vi "update event timing.vi"(4 "update duration":bool, 6 "Duration (s)":dbl, 8 "Start Time":timestamp format="%<%x %.3X>T", 9 "set start to now":bool, 10 "update start":bool, 11 "event":refnum<class "event.lvclass">) -> (0 "error out":errorcluster, 3 "updated event":refnum<class "event.lvclass">)   [LabVIEW 2020, in "nominal core steps.lvlib"]
doc: "Change the start time and duration of the event. Use flags to indicate which actions to take."
uses:
  nominal core steps.lvlib
  <vilib>/Nominal/Nominal IO Client/lv_src/event/event.lvclass
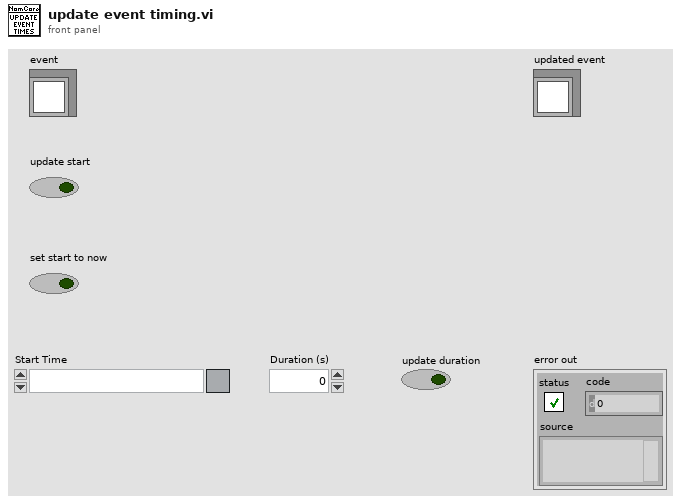
[diagram p1: front panel]
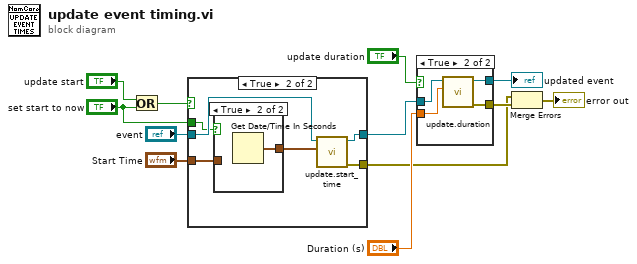
[diagram p0: block diagram]
diagram:
  n1 = Or(x="update start", y="set start to now") -> (x .or. y?=w2:bool)
  n2 = case shown="True" w2 {
    tunnel: [w13 w19] -> w6
    tunnel: [_ w18] -> w7
    tunnel: "event" -> [w13 w17]
    tunnel: "Start Time" -> [_ w14]
    tunnel: "set start to now" -> [_ w16]
    frame False {
    }
    frame True {
      n3 = case shown="True" w16 {
        tunnel: [w20 w21] -> w15
        tunnel: w14 -> [w20 _]
        frame False {
        }
        frame True {
          n4 = Get Date/Time In Seconds() -> (seconds since 1Jan1904=w21:timestamp)
        }
      }
      n5 = call <vilib>:"update.start_time.vi"("Start Time (empty: now)"=w15, "event in"=w17) -> ("error out"=w18:errorcluster, "event out"=w19:refnum<class "event.lvclass">)  [unwired: 8 in]
    }
  }
  n6 = case shown="True" "update duration" {
    tunnel: [_ w26] -> w8
    tunnel: [w22 w25] -> w4
    tunnel: "Duration (s)" -> [_ w24]
    tunnel: w6 -> [w22 w23]
    frame False {
    }
    frame True {
      n7 = call <vilib>:"update.duration.vi"("Duration (s)"=w24, "event in"=w23) -> ("error out"=w26:errorcluster, "event out"=w25:refnum<class "event.lvclass">)  [unwired: 8 in]
    }
  }
  "updated event" <- w4
  n8 = Merge Errors(w7, w8) -> (→"error out":errorcluster)
